vi "MQTT Client - Create.vi"(0 "Version (3.11)":T2=4 items=["3.11"=4, "5.0"=5], 1 "TCP Timeout (3000 ms)":i32=3000, 5 "Host":string="localhost", 7 "Port (1883)":u16=1883, 9 "Keep Alive (60 s)":u16=60, 11 "error in (no error)":errorcluster) -> (4 "MQTT Session":T1, 15 "error out":errorcluster)   [LabVIEW 2019, in "KoRE-MQTT.lvlib"]
doc: "<b>Description:</b> This VI prepares an MQTT client session by configuring the initial connection parameters. It does not establish a connection but provides a session reference for further configuration with <b>MQTT Client - Configure ???.vi<b> (e.g. Auth, TLS and Will) before connecting with <b>MQTT Client - Connect.vi</b>.\n\n<b>Input Terminals:</b>\n- <b>TCP Timeout (3000 ms) [1]</b>: The maximum time (in milliseconds) to wait for a TCP connections to respond before timing out. Default is 3000 ms.\n- <b>Version (3.11) [0]</b>: The MQTT protocol version to use for the session. Default is version 3.11.\n- <b>Host [5]</b>: The hostname or IP address of the MQTT broker to connect to.\n- <b>Port (1883) [7]</b>: The port number on which the MQTT broker is listening. Default is 1883, commonly used for non-secure MQTT connections. The standard default port for secure MQTT connections using TLS is **8883**.\n- <b>Keep Alive (60 s) [9]</b>: The duration (in seconds) to wait before sending a keep-alive message to the broker. Default is 60 seconds.\n\n<b>Output Terminals:</b>\n- <b>MQTT Session [4]</b>: Reference to the prepared MQTT client session, which can be further configured before connecting to the broker.\n\n\nCopyright (c) 2025 KoRElibs.com\nSPDX-License-Identifier: EUPL-1.2\n\nThis VI is licensed under the European Union Public License (EUPL) Version 1.2. You may use this VI unmodified in proprietary works. If you distribute a modified version of this file, the modified file must be released under the EUPL-1.2. Full license: https://joinup.ec.europa.eu/asset/eupl/eupl/1.2/"
uses:
  KoRE-MQTT.lvlib
  TypeDefs/MQTT Version.ctl
  TypeDefs/MQTT Client Session.ctl
  TypeDefs/MQTT Client Session - Data.ctl
  TypeDefs/MQTT Property - Will.ctl
  TypeDefs/MQTT Property - CONNECT.ctl
  Private/TypeDefs/MQTT Subscription - Info.ctl
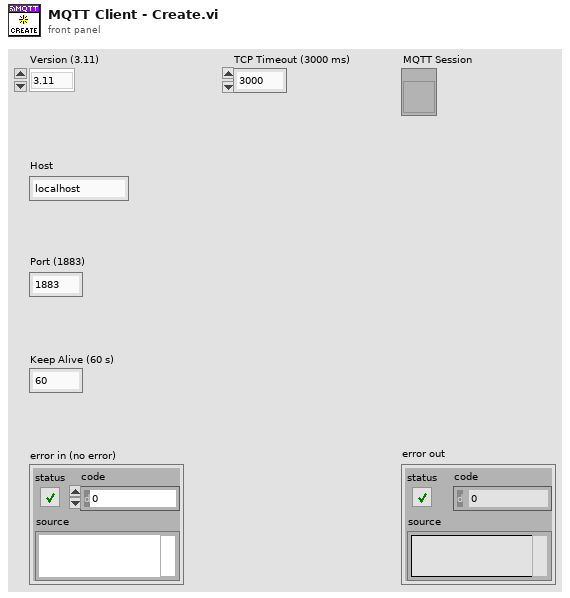
[diagram p1: front panel]
types:
  T1 = typedef "KoRE-MQTT.lvlib/MQTT Client Session.ctl" = refnum<vi>
  T2 = typedef "KoRE-MQTT.lvlib/MQTT Version.ctl" = u16
  T3 = typedef "KoRE-MQTT.lvlib/MQTT Client Session - Data.ctl" = cluster{"TCP ref":refnum<k5>, "Next Packet Id":u16, "Version":u8, "Host":string, "Port":u16, "Ping Delta":u32, "Username":string, "Password":string, "Will QoS":u8, "Will Retain":bool, "Will Topic":string, "Will Payload":string, "TCP Timeout":i32, "Semaphore":T4, "In-Flight Messages":variant, "Close":bool, "Last Send":u32, "Keep Alive":u16, "Last Ping RTT":u32, "Last Ping":u32, "Will Properties":T5[], "Session Expiry Interval":u32, "Maximum QoS":u8, "Retain Available":bool, "Server Maximum Packet Size":u32, "Client Identifier":string, "Server Topic Alias Maximum":u16, "Wildcard Subscription Available":bool, "Subscription Identifier Available":bool, "Shared Subscription Available":bool, "Connect Properties":T6[], "Client Maximum Packet Size":u32, "Client Topic Alias Maximum":u16, "Server Receive Maximum":u16, "Client Receive Maximum":u16, "TLS cfg":refnum<k36>, "Subscriptions":T7[]}
  T4 = typedef "Semaphore RefNum" = refnum<k1>
  T5 = typedef "KoRE-MQTT.lvlib/MQTT Property - Will.ctl" = cluster{"Property":u8, "Value":string}
  T6 = typedef "KoRE-MQTT.lvlib/MQTT Property - CONNECT.ctl" = cluster{"Property":u8, "Value":string}
  T7 = typedef "KoRE-MQTT.lvlib/MQTT Subscription - Info.ctl" = cluster{"Packet Id":u16, "Index":u16, "Identifier":u32, "QoS":u8, "Topic Filter":string, "Reason Code":u8, "Reason String":string, "Granted":bool}
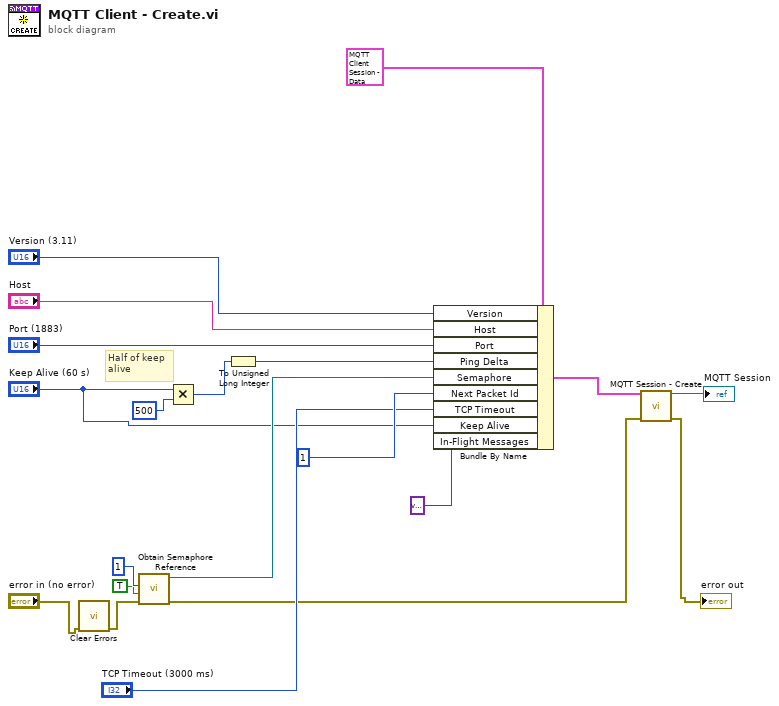
[diagram p0: block diagram]
diagram:
  # "Half of keep\nalive"
  n1 = call <vilib>:"Clear Errors.vi"("error in (no error)"="error in (no error)") -> ("error out"=w1:errorcluster)  [unwired: 5 in, 1 out]
  n2 = call <vilib>:"Obtain Semaphore Reference.vi"("error in (no error)"=w1, "create if not found (T)"=TRUE, "size (1)"=1) -> ("error out"=w4:errorcluster, "semaphore"=w16:T4)  [unwired: 2 in, 1 out]
  n3 = Multiply(x="Keep Alive (60 s)", y=u16 500) -> (x*y=w12:u16)
  n4 = To Unsigned Long Integer(number=w12) -> (unsigned 32bit integer=w10:u32)
  n5 = Bundle By Name(cluster=T3 {"TCP ref"=refnum, "Next Packet Id"=0, "Version"=0, "Host"="localhost", "Port"=1883, "Ping Delta"=60, "Username"="", "Password"="", "Will QoS"=0, "Will Retain"=FALSE, "Will Topic"="", "Will Payload"="", "TCP Timeout"=1000, "Semaphore"=refnum, "In-Flight Messages"=variant, "Close"=FALSE, "Last Send"=0, "Keep Alive"=0, "Last Ping RTT"=0, "Last Ping"=0, "Will Properties"=[], "Session Expiry Interval"=0, "Maximum QoS"=2, "Retain Available"=FALSE, "Server Maximum Packet Size"=0, "Client Identifier"="", "Server Topic Alias Maximum"=0, "Wildcard Subscription Available"=FALSE, "Subscription Identifier Available"=FALSE, "Shared Subscription Available"=FALSE, "Connect Properties"=[], "Client Maximum Packet Size"=0, "Client Topic Alias Maximum"=0, "Server Receive Maximum"=0, "Client Receive Maximum"=0, "TLS cfg"=refnum, "Subscriptions"=[]} ("Cluster"), "Version"="Version (3.11)", "Host"="Host", "Port"="Port (1883)", "Ping Delta"=w10, "Semaphore"=w16, "Next Packet Id"=u16 1 ("NextPacketId"), "TCP Timeout"="TCP Timeout (3000 ms)", "Keep Alive"="Keep Alive (60 s)", "In-Flight Messages"=variant ("QoS Lookup Table")) -> (w20:T3)
  n6 = call "MQTT Session - Create.vi"("mqtt config"=w20, "error in (no error)"=w4) -> ("mqtt ref"=→"MQTT Session":T1, "error out"=→"error out":errorcluster)  [unwired: 12 in]
